vi "Test Rename State.vi"(8 "error in (no error)":errorcluster) -> (0 "error out":errorcluster)   [LabVIEW 2020, in "TEST JKI State Machine API.lvlib"]
uses:
  TEST JKI State Machine API.lvlib
  source/JKI SM/JKI SM.lvclass
  <vilib>/addons/_JKI Toolkits/Caraya/classes/Test/Test.lvclass
  <vilib>/addons/_JKI Toolkits/Caraya/classes/Assert/Assert.lvclass
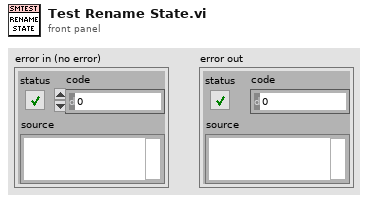
[diagram p1: front panel]
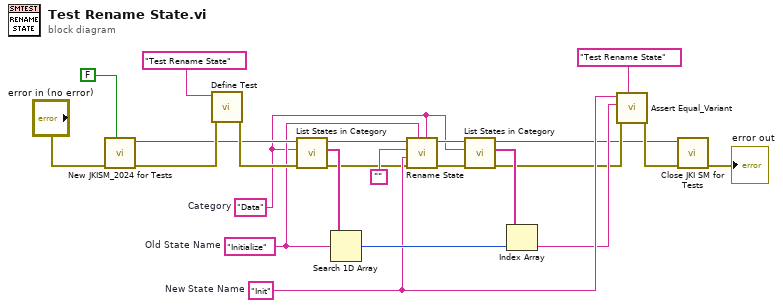
[diagram p0: block diagram]
diagram:
  w7 = "Init"  # New State Name
  w13 = "Initialize"  # Old State Name
  w10 = "Data"  # Category
  n1 = call "New JKISM_2024 for Tests.vi"("Open SM FP (for debugging)"=FALSE, "error in (no error)"="error in (no error)") -> ("error out"=w17:errorcluster, "JKI SM out"=w16:refnum<class "JKI SM.lvclass">)  [unwired: 8 in]
  n2 = call <vilib>:"Define Test.vi"("error in (no error)"=w17, "Label (VI Title)"="Test Rename State") -> ("error out"=w23:errorcluster)  [unwired: 8 in, 1 out]
  n3 = call "List States in Category.vi"("error in (no error)"=w23, "Category"=w10, "JKI SM in"=w16) -> ("error out"=w2:errorcluster, "States"=w15:string[], "JKI SM out"=w14:refnum<class "JKI SM.lvclass">)  [unwired: 4 in, 2 out]
  n4 = Search 1D Array(1D array=w15, element=w13) -> (index of element=w8:i32)  [unwired: 1 in]
  n5 = call-dynamic "Rename State.vi"("Category"=w10, "State"=w13, "error in (no error)"=w2, "New State"=w7, "New Category (\"\": Use Existing)"="" ("New Category (\"\": Use Existing)"), "JKI SM in"=w14) -> ("error out"=w12:errorcluster, "JKI SM out"=w11:refnum<class "JKI SM.lvclass">)  [unwired: 2 in, 2 out]
  n6 = call "List States in Category.vi"("error in (no error)"=w12, "Category"=w10, "JKI SM in"=w11) -> ("error out"=w5:errorcluster, "States"=w9:string[], "JKI SM out"=w4:refnum<class "JKI SM.lvclass">)  [unwired: 4 in, 2 out]
  n7 = Index Array(array=w9, index=w8) -> (element=w6:string)
  n8 = call <vilib>:"Assert Equal_Variant.vi"("Label"="Test Rename State", "error in (no error)"=w5, "Y"=w6, "X"=w7) -> ("error out"=w20:errorcluster)  [unwired: 7 in]
  n9 = call "Close JKI SM for Tests.vi"("error in (no error)"=w20, "JKI SM in"=w4) -> ("error out"=→"error out":errorcluster)  [unwired: 9 in]
